vi "Execute Job (Sync).vi"(8 "error in (no error)":errorcluster, 10 "stdin":string, 11 "Job in":refnum<class "Job.lvclass">) -> (0 "error out":errorcluster, 1 "JobReport":refnum<class "JobReport.lvclass">, 2 "stdout":string, 3 "Job out":refnum<class "Job.lvclass">)   [LabVIEW 2013, in "openCronJob.lvlib" / "Job.lvclass"]
uses:
  Job.lvclass
  JobReport/JobReport.lvclass
  Job.lvclass/Job.ctl
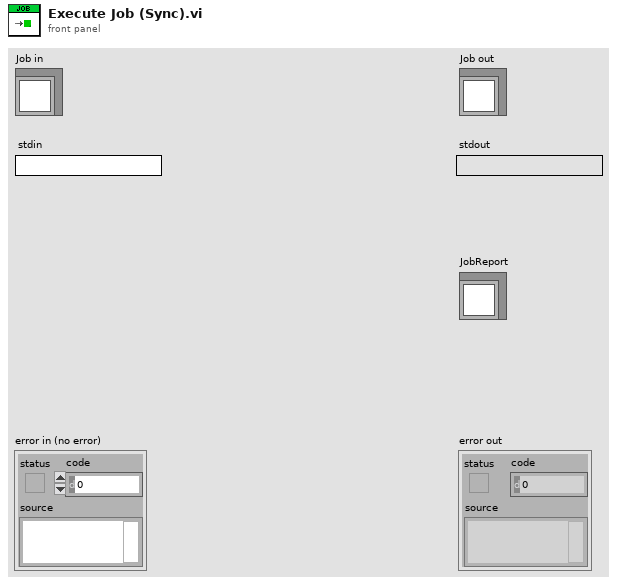
[diagram p1: front panel]
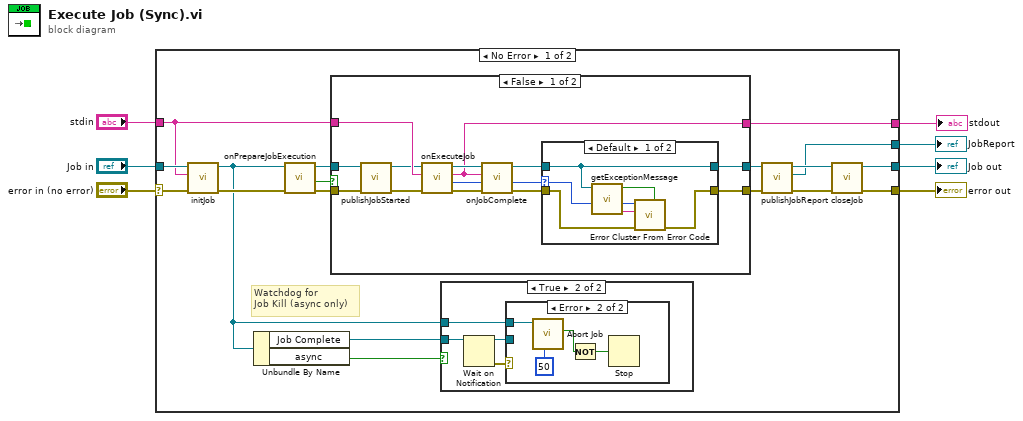
[diagram p0: block diagram]
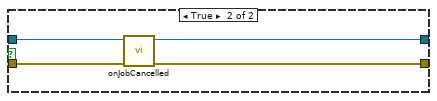
[diagram p5: hidden frame]
diagram:
  n1 = case shown="No Error" "error in (no error)" {
    selector: "error in (no error)" -> [w21 w62]
    tunnel: [w15 w61] -> w7
    tunnel: [w16 w62] -> w6
    tunnel: "Job in" -> [w22 w61]
    tunnel: [w8 _] -> w3
    tunnel: "stdin" -> [w14 _]
    tunnel: [w13 _] -> w1
    frame No Error {
      # "Watchdog for\nJob Kill (async only)"
      n2 = call "initJob.vi"("error in (no error)"=w21, "stdin"=w14, "Job in"=w22) -> ("error out"=w20:errorcluster, "Job out"=w17:refnum<class "Job.lvclass">)  [unwired: 7 in]
      n3 = Unbundle By Name(w17) -> ("Job Complete"=w18:refnum<notifier>, "async"=w19:bool)
      n4 = call-dynamic "onPrepareJobExecution.vi"("error in (no error)"=w20, "Job in"=w17) -> ("error out"=w24:errorcluster, "execution cancelled"=w23:bool, "Job out"=w25:refnum<class "Job.lvclass">)  [unwired: 7 in]
      n5 = case shown="False" w23 {
        tunnel: w25 -> [w37 w60]
        tunnel: w24 -> [w35 w59]
        tunnel: [w40 w57] -> w11
        tunnel: [w41 w58] -> w9
        tunnel: w14 -> [w39 _]
        tunnel: [w38 _] -> w13
        frame False {
          n6 = call "publishJobStarted.vi"("error in (no error)"=w35, "Job in"=w37) -> ("error out"=w34:errorcluster, "Job out"=w36:refnum<class "Job.lvclass">)  [unwired: 8 in]
          n7 = call-dynamic "onExecuteJob.vi"("error in (no error)"=w34, "stdin"=w39, "Job in"=w36) -> ("error out"=w46:errorcluster, "exception"=w45:i32, "stdout"=w38:string, "Job out"=w47:refnum<class "Job.lvclass">)  [unwired: 5 in]
          n8 = call-dynamic "onJobComplete.vi"("error in (no error)"=w46, "exception"=w45, "stdout"=w38, "Job in"=w47) -> ("error out"=w43:errorcluster, "unhandled exception"=w42:i32, "Job out"=w44:refnum<class "Job.lvclass">)  [unwired: 5 in]
          n9 = case shown="Default" w42 {
            selector: w42 -> [w52 _]
            tunnel: w43 -> [w54 w55]
            tunnel: w44 -> [w50 w56]
            tunnel: [w50 w56] -> w40
            tunnel: [w53 w55] -> w41
            frame Default {
              n10 = call-dynamic "getExceptionMessage.vi"("exception"=w52, "Job in"=w50) -> ("exception message"=w49:string, "exception dup"=w51:i32, "warning?"=w48:bool)  [unwired: 7 in]
              n11 = call <vilib>:"Error Cluster From Error Code.vi"("is warning? (False)"=w48, "error in (no error)"=w54, "error message (\"\")"=w49, "error code (0)"=w51) -> ("error out"=w53:errorcluster)  [unwired: 5 in]
            }
            frame 0 {
            }
          }
        }
        frame True {
          n12 = call-dynamic "onJobCancelled.vi"("error in (no error)"=w59, "Job in"=w60) -> ("error out"=w58:errorcluster, "Job out"=w57:refnum<class "Job.lvclass">)  [unwired: 8 in]
        }
      }
      n13 = case shown="True" w19 {
        tunnel: w18 -> [_ w29]
        tunnel: w17 -> [_ w26]
        frame False {
        }
        frame True {
          n14 = Wait on Notification(notifier=w29) -> (notifier out=w27:refnum<notifier>, error out=w28:errorcluster)  [unwired: 3 in, 2 out]
          n15 = case shown="Error" w28 {
            tunnel: w27 -> [_ _]
            tunnel: w26 -> [_ w33]
            frame No Error {
            }
            frame Error {
              n16 = call "Abort Job.vi"("timeout (500 ms)"=50, "Job in"=w33) -> ("Job Aborted"=w31:bool)  [unwired: 5 in, 4 out]
              n17 = Not(x=w31) -> (.not. x?=w30:bool)
              n18 = Stop(stop? (T)=w30) -> ()
            }
          }
        }
      }
      n19 = call "publishJobReport.vi"("error in (no error)"=w9, "Job in"=w11) -> ("error out"=w10:errorcluster, "JobReport"=w8:refnum<class "JobReport.lvclass">, "Job out"=w12:refnum<class "Job.lvclass">)  [unwired: 7 in]
      n20 = call "closeJob.vi"("error in (no error)"=w10, "Job in"=w12) -> ("error out"=w16:errorcluster, "Job out"=w15:refnum<class "Job.lvclass">)  [unwired: 8 in]
    }
    frame Error {
    }
  }
  "error out" <- w6
  "Job out" <- w7
  "JobReport" <- w3
  "stdout" <- w1
